vi "work2 _Cooker Module.vi"() -> ()   [LabVIEW 2026]
panel:
  in  "Nb burgers":u16
  in  "Burgers":bool
  in  "Meal":bool
  in  "stop":bool
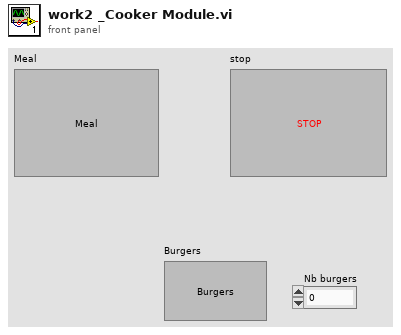
[diagram p1: front panel]
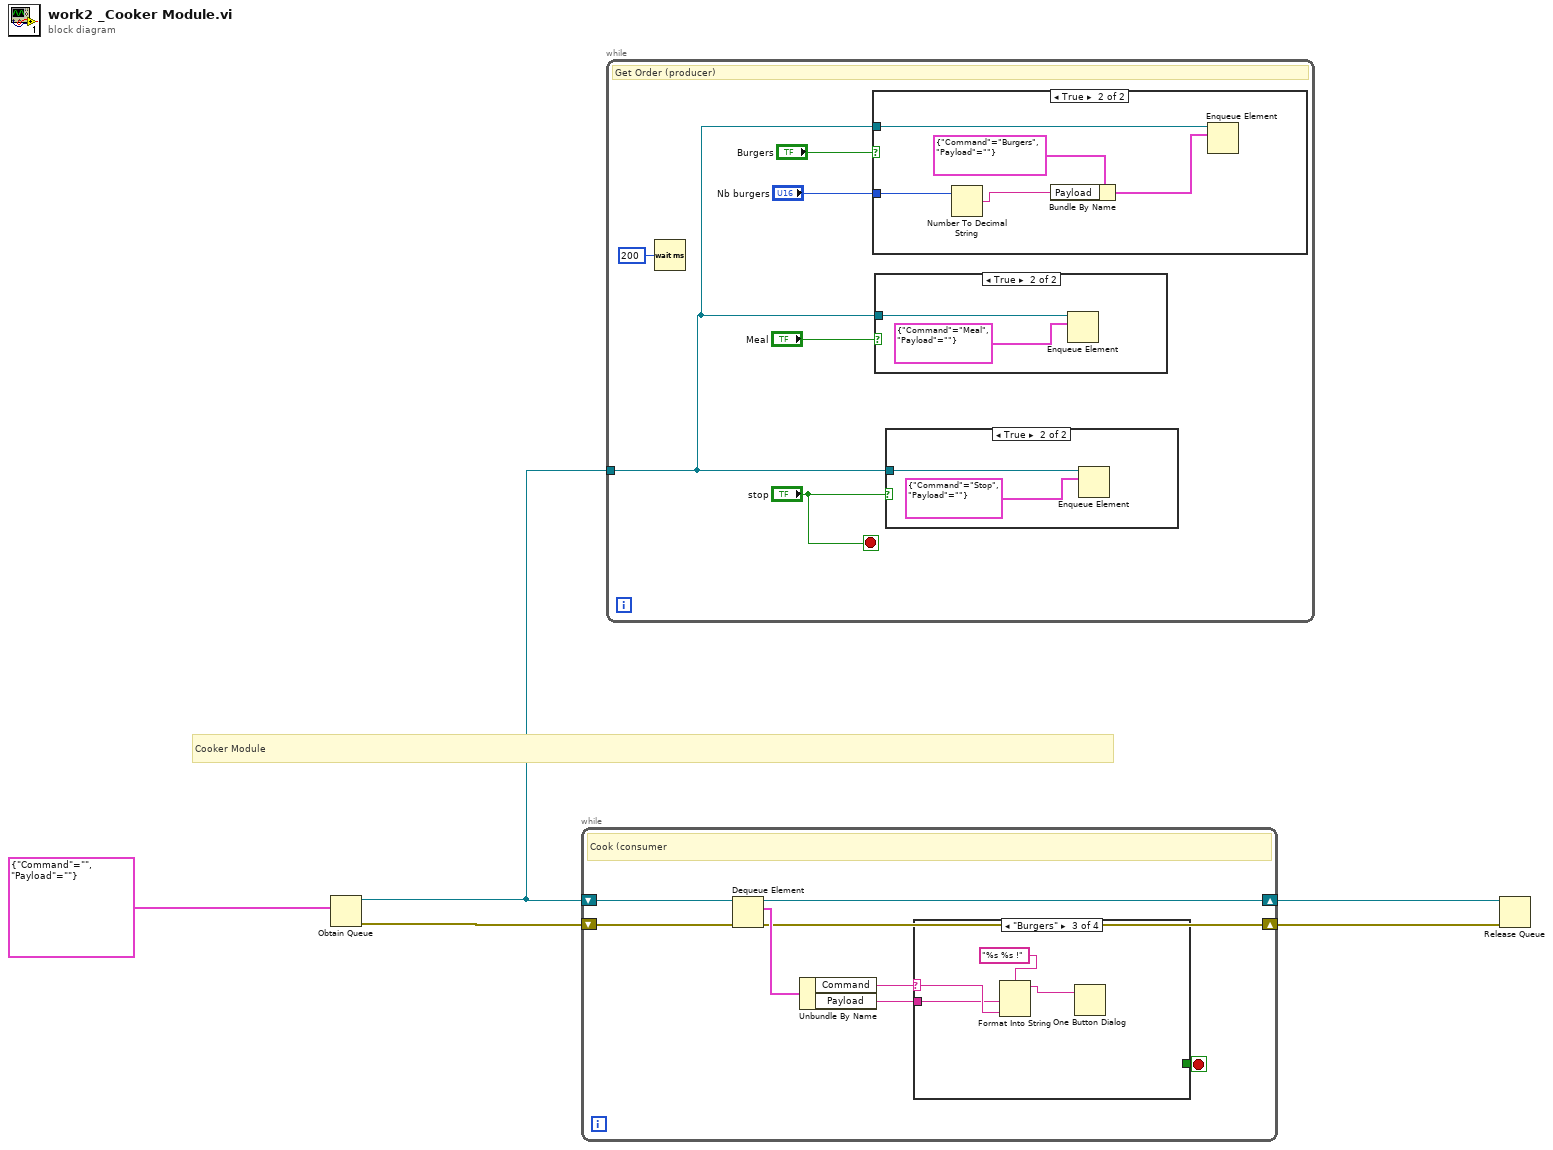
[diagram p0: block diagram]
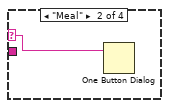
[diagram p6: hidden frame]
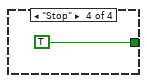
[diagram p7: hidden frame]
diagram:
  # "Cooker Module"
  n1 = Obtain Queue(element data type=cluster{"Command":string, "Payload":string} {"Command"="", "Payload"=""}) -> (queue out=w2:refnum<queue>, error out=w5:errorcluster)  [unwired: 4 in, 1 out]
  n2 = while {
    shift-right: [w8] -> w3
    shift-left: w5 -> [w13]
    shift-right: [w12] -> w4
    shift-left: w2 -> [w11]
    stop <- w7 stop-if-true
    # "Cook (consumer"
    n3 = Dequeue Element(queue=w11, error in (no error)=w13) -> (queue out=w12:refnum<queue>, element=w10:cluster{"Command":string, "Payload":string}, error out=w8:errorcluster)  [unwired: 1 in, 1 out]
    n4 = Unbundle By Name(w10) -> ("Command"=w9:string, "Payload"=w6:string)
    n5 = case shown="\"Burgers\"" w9 {
      selector: w9 -> [_ w14 w16 _]
      tunnel: [_ _ _ TRUE] -> w7
      tunnel: w6 -> [_ _ w15 _]
      frame "False", Default {
      }
      frame "Meal" {
        n6 = One Button Dialog(message=w14) -> ()  [unwired: 1 in, 1 out]
      }
      frame "Burgers" {
        n7 = Format Into String(format string="%s %s !", w15, w16) -> (resulting string=w17:string)  [unwired: 2 in, 1 out]
        n8 = One Button Dialog(message=w17) -> ()  [unwired: 1 in, 1 out]
      }
      frame "Stop" {
      }
    }
  }
  n9 = while {
    tunnel: w2 -> [w21]
    stop <- "stop" stop-if-true
    # "Get Order (producer)"
    n10 = Wait (ms)(milliseconds to wait=u32 200) -> ()  [unwired: 1 out]
    n11 = case shown="True" "Burgers" {
      tunnel: w21 -> [_ w30]
      tunnel: "Nb burgers" -> [_ w29]
      frame False {
      }
      frame True {
        n12 = Number To Decimal String(number=w29) -> (decimal integer string=w26:string)  [unwired: 1 in]
        n13 = Bundle By Name(cluster=cluster{"Command":string, "Payload":string} {"Command"="Burgers", "Payload"=""} ("element"), "Payload"=w26) -> (w27:cluster{"Command":string, "Payload":string})
        n14 = Enqueue Element(queue=w30, element=w27) -> ()  [unwired: 2 in, 3 out]
      }
    }
    n15 = case shown="True" "Meal" {
      tunnel: w21 -> [_ w32]
      frame False {
      }
      frame True {
        n16 = Enqueue Element(queue=w32, element=cluster{"Command":string, "Payload":string} {"Command"="Meal", "Payload"=""}) -> ()  [unwired: 2 in, 3 out]
      }
    }
    n17 = case shown="True" "stop" {
      tunnel: w21 -> [_ w34]
      frame False {
      }
      frame True {
        n18 = Enqueue Element(queue=w34, element=cluster{"Command":string, "Payload":string} {"Command"="Stop", "Payload"=""}) -> ()  [unwired: 2 in, 3 out]
      }
    }
  }
  n19 = Release Queue(queue=w4, error in (no error)=w3) -> ()  [unwired: 1 in, 3 out]
